vi "test13-AsteriskWildcardStateRegistration.vi"(8 "error in (no error)":errorcluster, 11 "TestCase in":refnum<class "testcase-CSMBroadcast.lvclass">) -> (0 "error out":errorcluster, 3 "TestCase out":refnum<class "testcase-CSMBroadcast.lvclass">)   [LabVIEW 2017, in "testcase-CSMBroadcast.lvclass"]
uses:
  testcase-CSMBroadcast.lvclass
  0c20cacf-7d77-4f8e-aec5-f22e7d09936d.vi
  2ac2ae3e-7b57-4584-ae51-4de7b8fb2940.vi
  26de337d-8090-412f-9da5-e117a55d4726.vi
  de10340a-d592-45ad-b055-7fa7b377c551.vi
  e3eae2f8-d8ce-4adb-8167-9a417250fce1.vi
  a4d00e00-a9ed-4631-bf53-269bf71f16fc.vi
  src/user.lib/_NEVSTOP/Communicable State Machine(CSM)/AdvanceAPI/CSM - Revert Arguments-Safe String.vi
  src/user.lib/_NEVSTOP/Communicable State Machine(CSM)/_Shared/Trim Single-line Text.vi
  src/user.lib/_NEVSTOP/Communicable State Machine(CSM)/AdvanceAPI/CSM - Make String Arguments Safe.vi
  src/user.lib/_NEVSTOP/Communicable State Machine(CSM)/AdvanceAPI/CSM - Break Down Multiple States String.vi
  src/user.lib/_NEVSTOP/Communicable State Machine(CSM)/AdvanceAPI/CSM - Compact Multiple States.vi
  src/user.lib/_NEVSTOP/Communicable State Machine(CSM)/AdvanceAPI/CSM - Keywords.vi
  src/user.lib/_NEVSTOP/Communicable State Machine(CSM)/AdvanceAPI/CSM - Set Module Attribute.vi
  src/user.lib/_NEVSTOP/Communicable State Machine(CSM)/AdvanceAPI/CSM - Get Module Attribute.vi
  <vilib>/addons/_JKI Toolkits/VI Tester/TestCase.llb/TestCase.lvclass
  src/user.lib/_NEVSTOP/Communicable State Machine(CSM)/Communicable State Machine.lvlib
  C:/Program Files (x86)/National Instruments/LabVIEW 2017/vi.lib/addons/_JKI Toolkits/VI Tester/TestCase.llb/TestCase.lvclass
panel:
  out "Execution Times":i32
  out "State History":string
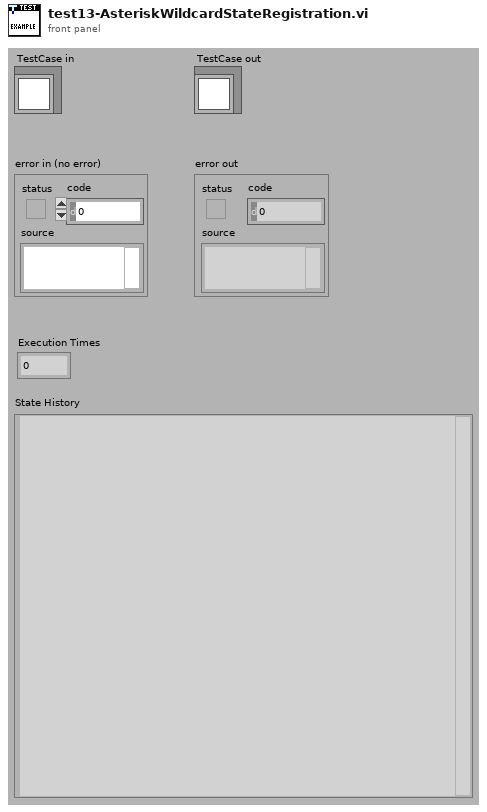
[diagram p1: front panel]
types:
  T1 = enum32{"Invalid", "Standard", "Closed", "Hidden", "Minimized", "Maximized"}
  T2 = enum32{"invalid app kind", "Development System", "Run Time System", "Student Edition", "Embedded LabVIEW", "Evaluation", "Custom"}
  T3 = typedef "Communicable State Machine.lvlib/_CSM_Response Source Message.ctl" = cluster{"‘State":string, "’Arguments":string, "’Error":errorcluster}
  T4 = cluster{"Current VI Reference":refnum<vi>, "Close Panel on Exit?":bool}
  T5 = cluster{"Core":cluster{"Current VI Reference":refnum<vi>, "Close Panel on Exit?":bool}, "Your Boolean data":bool, "Your string data":string, "TestData":i32}
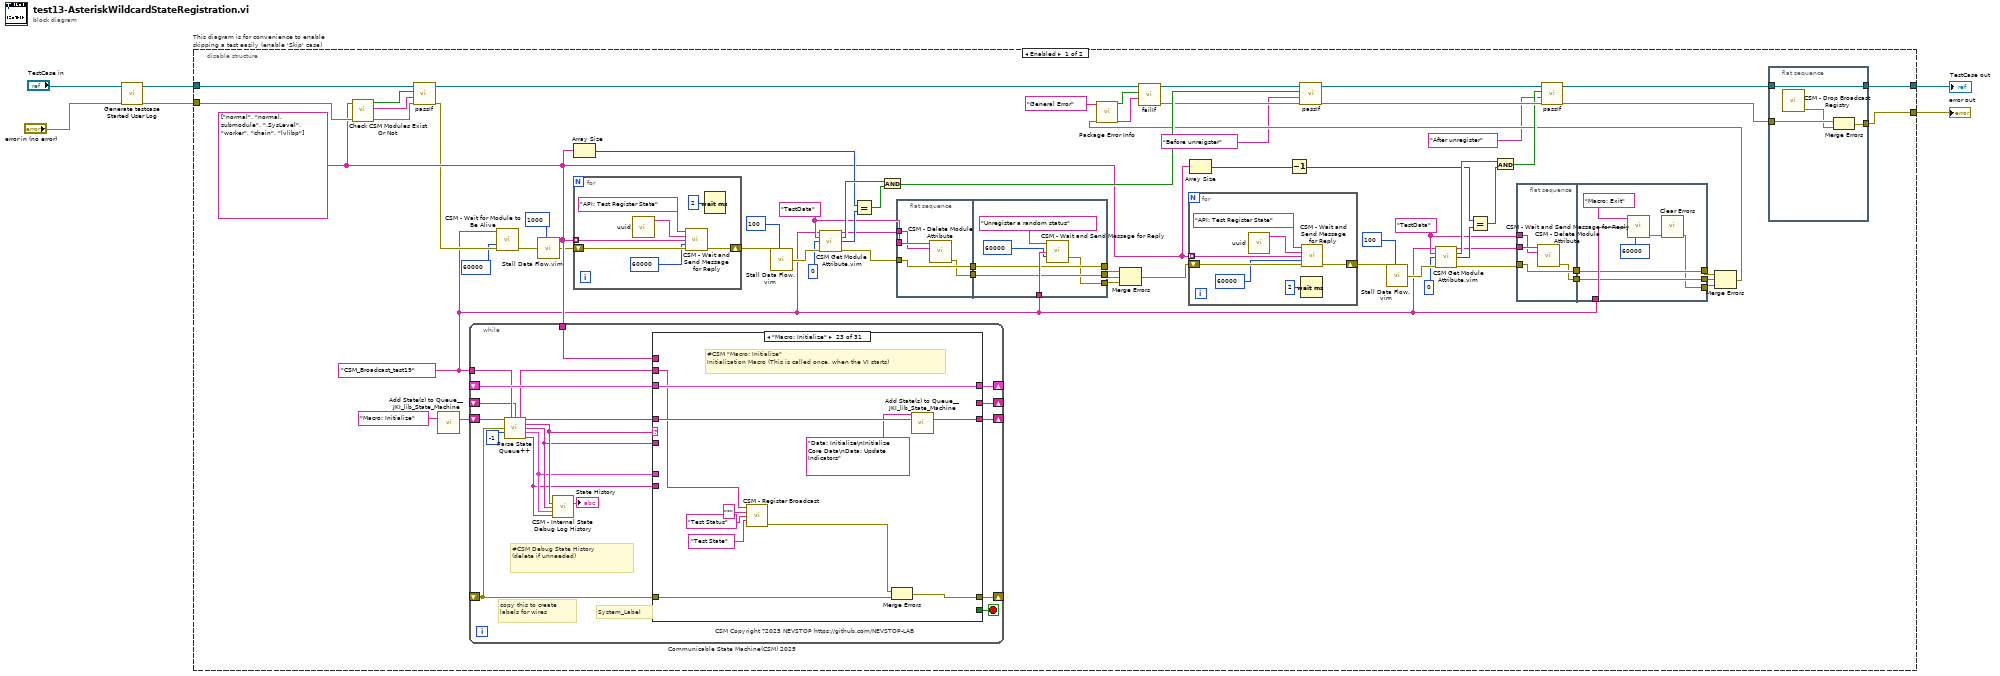
[diagram p0: block diagram]
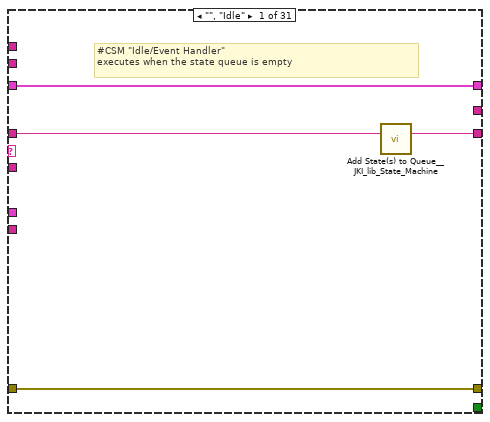
[diagram p2: hidden frame]
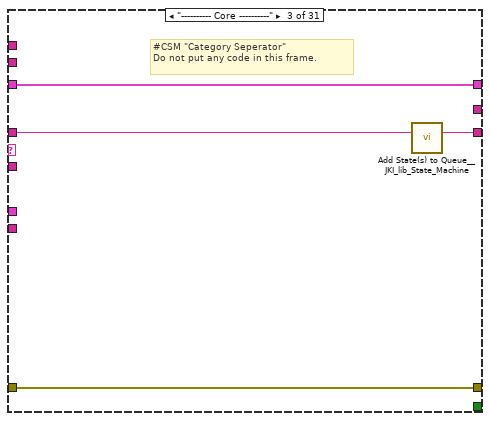
[diagram p4: hidden frame]
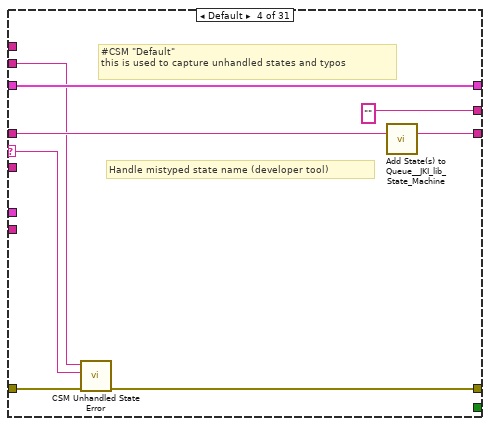
[diagram p5: hidden frame]
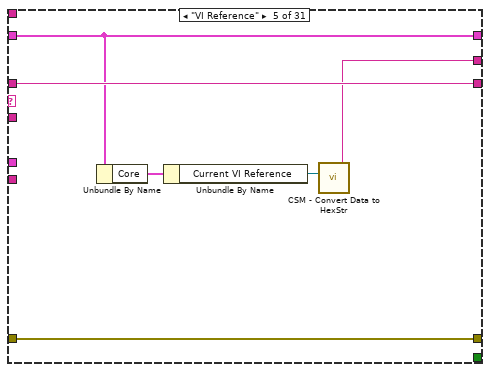
[diagram p6: hidden frame]
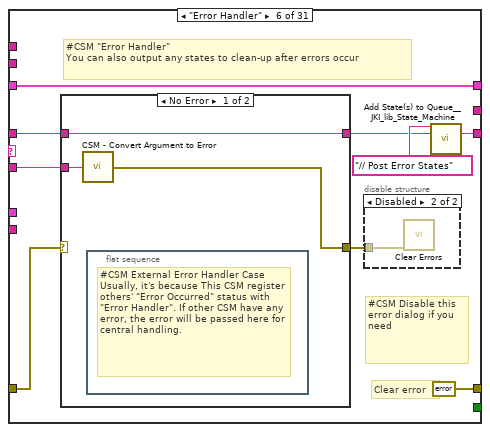
[diagram p7: hidden frame]
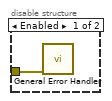
[diagram p8: hidden frame]
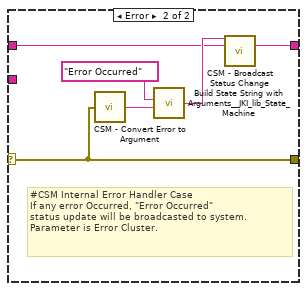
[diagram p9: hidden frame]
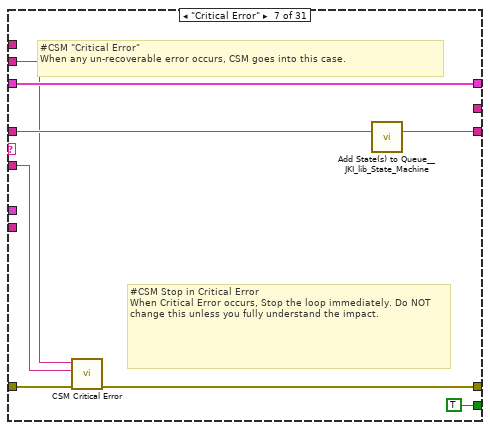
[diagram p10: hidden frame]
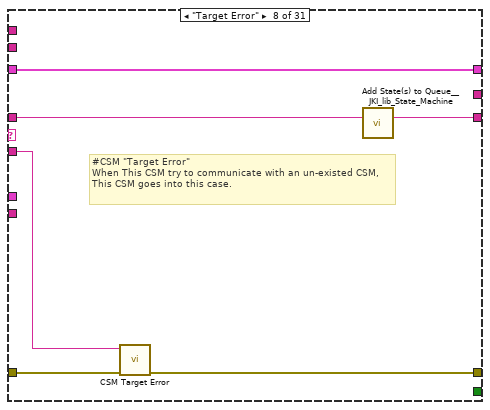
[diagram p11: hidden frame]
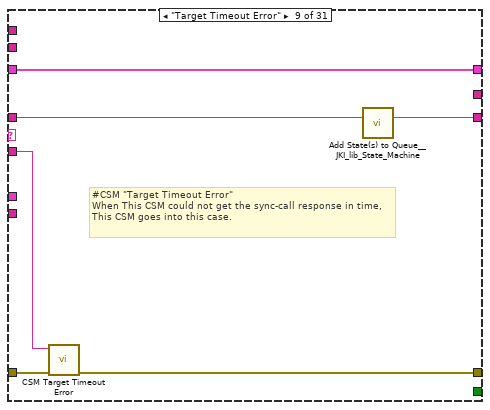
[diagram p12: hidden frame]
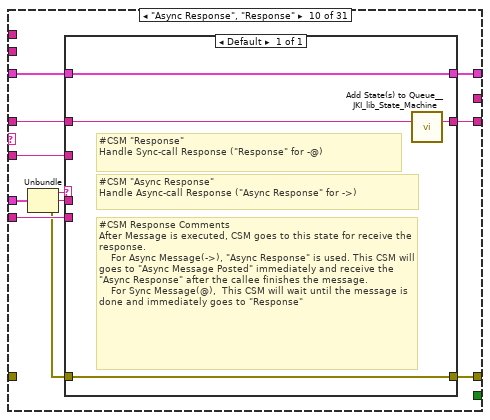
[diagram p13: hidden frame]
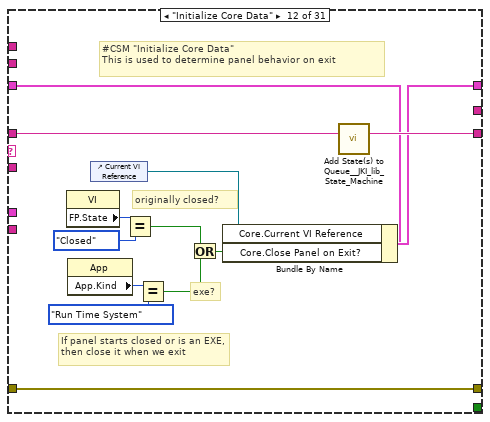
[diagram p15: hidden frame]
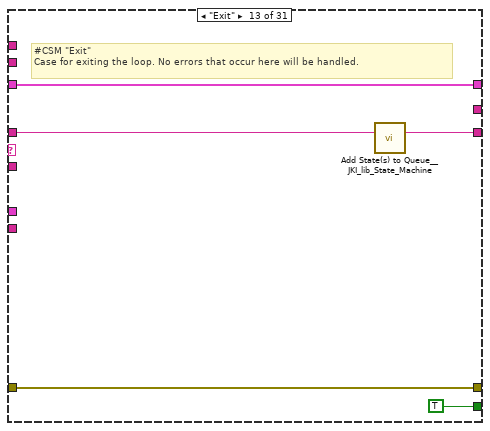
[diagram p16: hidden frame]
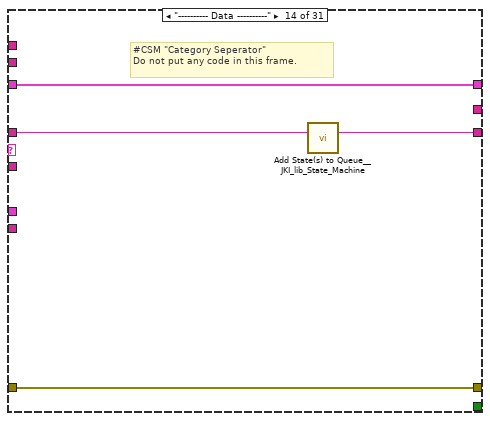
[diagram p17: hidden frame]
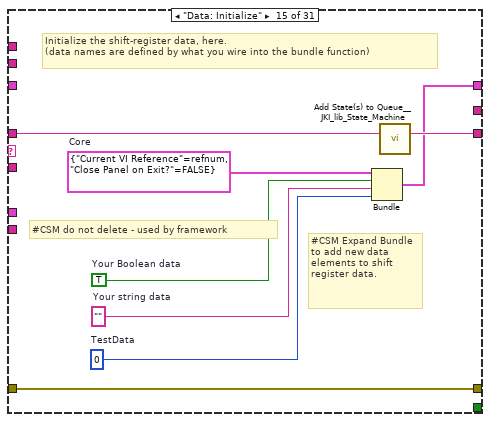
[diagram p18: hidden frame]
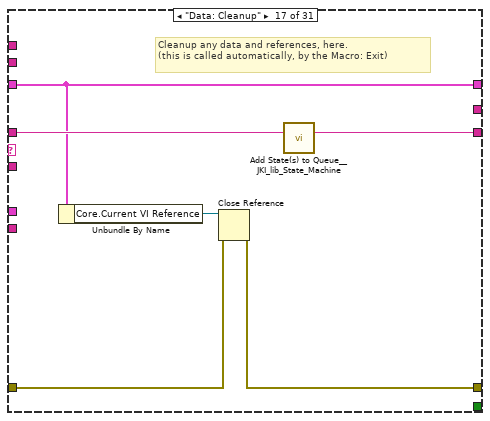
[diagram p20: hidden frame]
diagram:
  n1 = call "Generate testcase Started User Log.vi"("Error In"="error in (no error)") -> ("error out"=w1:errorcluster)  [unwired: 10 in]
  n2 = disable-structure "This diagram is for convenience to enable skipping a test easily (enable 'Skip' case)" shown="Enabled" {
    disable-tunnel: "TestCase in" -> [w27 w429]
    disable-tunnel: [w22 w427] -> w2
    disable-tunnel: [w21 w428] -> w4
    disable-tunnel: w1 -> [w26 w426]
    frame Enabled {
      w36 = "TestData" ("Attribute")
      w58 = "TestData" ("Attribute")
      w9 = "CSM_Broadcast_test19" ("Name (\"\" to Use UUID)")
      w25 = string[] ["normal", "normal.submodule", ".SysLevel", "worker", "chain", "lvlibp"]
      n3 = call "Check CSM Modules Exist Or Not.vi"("error in"=w26, "CSM names in"=w25) -> ("error out"=w28:errorcluster, "Debug string"=w29:string, "All Modules Exist?"=w30:bool)  [unwired: 7 in]
      n4 = call-dynamic "passIf.vi"("error in (no error)"=w28, "message (\"\")"=w29, "pass"=w30, "TestCase in"=w27) -> ("error out"=w10:errorcluster, "TestCase out"=w19:refnum<class "testcase-CSMBroadcast.lvclass">)  [unwired: 6 in]
      n5 = call <vilib>:"Add State(s) to Queue__JKI_lib_State_Machine.vi"("State(s) in (\"\")"="Macro: Initialize" ("Init State(\"Macro: Initialize\")")) -> ("States Out"=w69:string)  [unwired: 14 in]
      n6 = while "Communicable State Machine(CSM) 2025" {
        shift-right: [w116] -> _
        shift-left: _ -> [w115]
        shift-right: [w119] -> _
        shift-left: _ -> [w114]
        shift-right: [w118] -> _
        shift-left: w69 -> [w120]
        tunnel: w9 -> [w112]
        shift-right: [w113] -> _
        shift-left: _ -> [w106]
        tunnel: w25 -> [w103]
        stop <- w117 stop-if-true
        # "#CSM Debug State History\n(delete if unneeded)"
        # "copy this to create labels for wires"
        # "System_Label"
        # "CSM Copyright ?2025 NEVSTOP https://github.com/NEVSTOP-LAB"
        n7 = call "Parse State Queue++.vi"("State Queue"=w120, "Name (\"\" to Use UUID)"=w112, "Response Arguments"=w106, "Previous Error"=w114, "Dequeue (1 ms)"=-1 ("Timeout")) -> ("Name Used"=w107:string, "Remaining States"=w121:string, "Current State"=w111:string, "Arguments"=w110:string, "Additional Information"=w109:T3, "Source CSM"=w108:string)  [unwired: 5 in]
        n8 = call "CSM - Internal State Debug Log History.vi"("State"=w111, "Arguments (\"\")"=w110, ">> Response Source Message >>"=w109, "Source (\"\")"=w108) -> ("Debug Log"=→"State History":string)  [unwired: 11 in]
        n9 = case shown="\"Macro: Initialize\"" w111 {
          selector: w111 -> [_ _ _ w135 _ _ _ _ _ _ _ _ _ _ _ _ _ _ _ _ _ _ _ _ _ _ _ _ _ _ _]
          tunnel: w121 -> [w122 w127 w132 w139 w145 w151 w172 w178 w184 w192 w203 w217 w222 w226 w234 w236 w243 w247 w251 w257 w272 w341 w352 w365 w367 w371 w376 w383 w387 w398 w418]
          tunnel: w110 -> [_ _ _ _ _ w150 w168 w177 w182 w191 _ _ _ _ _ _ _ _ _ w252 w266 _ _ _ _ _ w374 _ _ _ _]
          tunnel: w115 -> [w123 w126 w129 w137 w144 w154 w173 w179 w185 w194 w202 w210 w220 w223 _ w235 w238 w244 w249 w255 w268 w338 w349 w362 w366 w370 w375 w380 w384 w390 w404]
          tunnel: [w124 w128 w130 w133 w146 errorcluster {"status"=FALSE, "code"=0, "source"=""} ("error out") w169 w175 w181 w197 w204 w214 w219 w224 w231 w237 w239 w245 w248 w253 w269 w339 w343 w354 w368 w372 w377 w381 w385 w392 w406] -> w119
          tunnel: w114 -> [w124 w128 w130 w140 w146 w152 w174 w176 w183 _ w204 w214 w219 w224 w231 w237 w240 w245 w248 w254 w270 w339 w350 w363 w368 w372 w377 w381 w385 w396 w416]
          tunnel: [w125 w127 w131 w138 w145 w147 w171 w180 w186 w193 w203 w216 w221 w225 w233 w236 w242 w246 w250 w256 w271 w340 w351 w364 w367 w371 w376 w382 w386 w397 w417] -> w118
          tunnel: [_ _ _ _ _ _ TRUE _ _ _ _ _ TRUE _ _ _ _ _ _ _ _ _ _ _ _ _ _ _ _ _ _] -> w117
          tunnel: [w123 w126 w129 w137 w144 w154 w173 w179 w185 w195 w202 w215 w220 w223 w232 w235 w238 w244 w249 w255 w268 w338 w349 w362 w366 w370 w375 w380 w384 w394 w402] -> w116
          tunnel: w108 -> [_ _ _ _ _ _ _ _ _ w189 _ _ _ _ _ _ _ _ _ _ _ _ _ _ _ _ _ _ _ _ _]
          tunnel: w109 -> [_ _ _ _ _ _ _ _ _ w196 _ _ _ _ _ _ _ _ _ _ _ _ _ _ _ _ _ _ _ _ _]
          tunnel: [_ _ _ "" w141 _ _ _ _ _ _ _ _ _ _ _ _ _ _ _ _ _ _ _ _ "API1 Response" w373 _ _ _ _] -> w113
          tunnel: w107 -> [_ _ _ w134 _ _ w167 _ _ _ _ _ _ _ _ _ _ _ _ _ _ _ w344 w356 _ _ _ _ _ w393 w413]
          tunnel: w103 -> [_ _ _ _ _ _ _ _ _ _ _ _ _ _ _ _ _ _ _ _ _ _ _ _ _ _ _ _ _ _ w409]
          frame "", "Idle" {
            # "#CSM \"Idle/Event Handler\"\nexecutes when the state queue is empty"
            n10 = call <vilib>:"Add State(s) to Queue__JKI_lib_State_Machine.vi"("State(s) in (\"\")"=w122) -> ("States Out"=w125:string)  [unwired: 14 in]
          }
          frame "CSM Documentation" {
            # "#CSM README FIRST\n\nCommunicable State Machine(CSM) is a LabVIEW application framework that builds upon JKI State Machine(JKISM). It follows the pattern of JKISM and extends the keywords to describe message communication between modules, including concepts such as Sync-Message, Async-Message, Subscription/Unsubscription of status - essential elements for creating reusable code modules. For more information, please visit the CSM wiki: https://nevstop-lab.github.io/CSM-Wiki/\n\nFor instructions on JKI State Machine, visit: http://jki.net/state-machine/\nFor information about CSM, visit: https://github.com/NEVSTOP-LAB"
            # "#CSM \"Documentation\"\nCase for holding CSM Documenation"
          }
          frame "---------- Core ----------" {
            # "#CSM \"Category Seperator\"\nDo not put any code in this frame."
            n11 = call <vilib>:"Add State(s) to Queue__JKI_lib_State_Machine.vi"("State(s) in (\"\")"=w132) -> ("States Out"=w131:string)  [unwired: 14 in]
          }
          frame Default {
            # "#CSM \"Default\"\nthis is used to capture unhandled states and typos"
            # "Handle mistyped state name (developer tool)"
            n12 = call "CSM Unhandled State Error.vi"("error in (no error)"=w140, "Undefined State"=w135, "CSM Name"=w134) -> ("error out"=w133:errorcluster)  [unwired: 8 in]
            n13 = call <vilib>:"Add State(s) to Queue__JKI_lib_State_Machine.vi"("State(s) in (\"\")"=w139) -> ("States Out"=w138:string)  [unwired: 14 in]
          }
          frame "VI Reference" {
            n14 = Unbundle By Name(w144) -> ("Core"=w143:T4)
            n15 = Unbundle By Name(w143) -> ("Current VI Reference"=w142:refnum<vi>)
            n16 = call "CSM - Convert Data to HexStr.vi"("Variant"=w142) -> ("HEX String (0-9,A-F)"=w141:string)  [unwired: 8 in]
          }
          frame "Error Handler" {
            # "#CSM Disable this error dialog if you need"
            # "#CSM \"Error Handler\"\nYou can also output any states to clean-up after errors occur"
            # "Clear error"
            n17 = case shown="No Error" w152 {
              selector: w152 -> [_ w161]
              tunnel: [w160 w163] -> w148
              tunnel: w151 -> [w160 w162]
              tunnel: w150 -> [w159 _]
              tunnel: [w158 w161] -> w153
              frame No Error {
                n18 = call "CSM - Convert Argument to Error.vi"("Argument"=w159) -> ("Error"=w158:errorcluster)  [unwired: 4 in]
                n19 = flat-sequence {
                  frame #0 {
                    # "#CSM External Error Handler Case\nUsually, it's because This CSM register others' \"Error Occurred\" status with \"Error Handler\". If other CSM have any error, the error will be passed here for central handling."
                  }
                }
              }
              frame Error {
                # "#CSM Internal Error Handler Case \nIf any error Occurred, \"Error Occurred\" \nstatus update will be broadcasted to system.\nParameter is Error Cluster."
                n20 = call "CSM - Convert Error to Argument.vi"("Error"=w161) -> ("Argument"=w165:string)  [unwired: 4 in]
                n21 = call <vilib>:"Build State String with Arguments__JKI_lib_State_Machine.vi"("Arguments (\"\")"=w165, "State"="Error Occurred" ("Status with Arguments")) -> ("State with Arguments"=w164:string)  [unwired: 4 in]
                n22 = call "CSM - Broadcast Status Change.vi"("Status With Arguments"=w164, "State Queue"=w162) -> ("Remaining States"=w163:string)  [unwired: 13 in]
              }
            }
            n23 = disable-structure shown="Disabled" {
              disable-tunnel: w153 -> [w156 w157]
              frame Enabled {
                n24 = call <vilib>:"General Error Handler.vi"("error in (no error)"=w156) -> ()  [unwired: 10 in, 5 out]
              }
              frame Disabled {
                n25 = call <vilib>:"Clear Errors.vi"("error in (no error)"=w157) -> ()  [unwired: 5 in, 2 out]
              }
            }
            n26 = call <vilib>:"Add State(s) to Queue__JKI_lib_State_Machine.vi"("State(s) in Front (\"\")"="// Post Error States", "State(s) in (\"\")"=w148) -> ("States Out"=w147:string)  [unwired: 13 in]
          }
          frame "Critical Error" {
            # "#CSM Stop in Critical Error\nWhen Critical Error occurs, Stop the loop immediately. Do NOT change this unless you fully understand the impact."
            # "#CSM \"Critical Error\"\nWhen any un-recoverable error occurs, CSM goes into this case."
            n27 = call "CSM Critical Error.vi"("error in (no error)"=w174, "Arugments (As Reason)"=w168, "CSM Name"=w167) -> ("error out"=w169:errorcluster)  [unwired: 8 in]
            n28 = call <vilib>:"Add State(s) to Queue__JKI_lib_State_Machine.vi"("State(s) in (\"\")"=w172) -> ("States Out"=w171:string)  [unwired: 14 in]
          }
          frame "Target Error" {
            # "#CSM \"Target Error\"\nWhen This CSM try to communicate with an un-existed CSM, This CSM goes into this case."
            n29 = call "CSM Target Error.vi"("error in (no error)"=w176, "Arguments (As CSM Name)"=w177) -> ("error out"=w175:errorcluster)  [unwired: 9 in]
            n30 = call <vilib>:"Add State(s) to Queue__JKI_lib_State_Machine.vi"("State(s) in (\"\")"=w178) -> ("States Out"=w180:string)  [unwired: 14 in]
          }
          frame "Target Timeout Error" {
            # "#CSM \"Target Timeout Error\"\nWhen This CSM could not get the sync-call response in time, This CSM goes into this case."
            n31 = call "CSM Target Timeout Error.vi"("error in (no error)"=w183, "Arguments (As CSM Name)"=w182) -> ("error out"=w181:errorcluster)  [unwired: 9 in]
            n32 = call <vilib>:"Add State(s) to Queue__JKI_lib_State_Machine.vi"("State(s) in (\"\")"=w184) -> ("States Out"=w186:string)  [unwired: 14 in]
          }
          frame "Async Response", "Response" {
            n33 = Unbundle(w196) -> ("‘State"=w190:string, "’Arguments"=w188:string, "’Error"=w187:errorcluster)
            n34 = case shown="Default" w190 {
              tunnel: [w201] -> w197
              tunnel: w187 -> [w201]
              tunnel: [w200] -> w195
              tunnel: w194 -> [w200]
              tunnel: [w198] -> w193
              tunnel: w192 -> [w199]
              tunnel: w191 -> [_]
              tunnel: w189 -> [_]
              tunnel: w188 -> [_]
              frame Default {
                # "#CSM Response Comments\nAfter Message is executed, CSM goes to this state for receive the response.\n    For Async Message(->), \"Async Response\" is used. This CSM will goes to \"Async Message Posted\" immediately and receive the \"Async Response\" after the callee finishes the message.\n    For Sync Message(@),  This CSM will wait until the message is done and immediately goes to \"Response\""
                # "#CSM \"Async Response\"\nHandle Async-call Response (\"Async Response\" for ->)"
                # "#CSM \"Response\"\nHandle Sync-call Response (\"Response\" for -@)"
                n35 = call <vilib>:"Add State(s) to Queue__JKI_lib_State_Machine.vi"("State(s) in (\"\")"=w199) -> ("States Out"=w198:string)  [unwired: 14 in]
              }
            }
          }
          frame "Async Message Posted" {
            # "#CSM \"Async Message Posted\"\nAfter Async Message is posted (-> or ->| ), CSM goes to this state for post-action.\nYou can use Argument - State to tell which Async Message is called."
          }
          frame "Initialize Core Data" {
            # "#CSM \"Initialize Core Data\"\nThis is used to determine panel behavior on exit"
            # "originally closed?"
            # "exe?"
            # "If panel starts closed or is an EXE, then close it when we exit"
            n36 = property class="VI"() -> ("FP.State"=w207:T1)  [unwired: 2 in, 2 out]
            n37 = property class="App"() -> ("App.Kind"=w213:T2)  [unwired: 2 in, 2 out]
            n38 = control-ref of="Current VI Reference"() -> (w208:refnum<vi>)
            n39 = Equal?(x=w207, y=T1."Closed" ("Front Panel Window:State")) -> (x = y?=w205:bool)
            n40 = Equal?(x=w213, y=T2."Run Time System" ("Application:Kind")) -> (x = y?=w211:bool)
            n41 = Or(x=w205, y=w211) -> (x .or. y?=w209:bool)
            n42 = Bundle By Name(cluster=w210, "Core.Current VI Reference"=w208, "Core.Close Panel on Exit?"=w209) -> (w215:T5)
            n43 = call <vilib>:"Add State(s) to Queue__JKI_lib_State_Machine.vi"("State(s) in (\"\")"=w217) -> ("States Out"=w216:string)  [unwired: 14 in]
          }
          frame "Exit" {
            # "#CSM \"Exit\"\nCase for exiting the loop. No errors that occur here will be handled."
            n44 = call <vilib>:"Add State(s) to Queue__JKI_lib_State_Machine.vi"("State(s) in (\"\")"=w222) -> ("States Out"=w221:string)  [unwired: 14 in]
          }
          frame "---------- Data ----------" {
            # "#CSM \"Category Seperator\"\nDo not put any code in this frame."
            n45 = call <vilib>:"Add State(s) to Queue__JKI_lib_State_Machine.vi"("State(s) in (\"\")"=w226) -> ("States Out"=w225:string)  [unwired: 14 in]
          }
          frame "Data: Initialize" {
            w227 = 0  # TestData
            w228 = T4 {"Current VI Reference"=refnum, "Close Panel on Exit?"=FALSE}  # Core
            w230 = TRUE  # Your Boolean data
            w229 = ""  # Your string data
            # "#CSM do not delete - used by framework"
            # "#CSM Expand Bundle to add new data elements to shift register data."
            # "Initialize the shift-register data, here.\n(data names are defined by what you wire into the bundle function)"
            n46 = Bundle("Core"=w228, "Your Boolean data"=w230, "Your string data"=w229, "TestData"=w227) -> (w232:T5)  [unwired: 1 in]
            n47 = call <vilib>:"Add State(s) to Queue__JKI_lib_State_Machine.vi"("State(s) in (\"\")"=w234) -> ("States Out"=w233:string)  [unwired: 14 in]
          }
          frame "Data: Update Indicators" {
          }
          frame "Data: Cleanup" {
            # "Cleanup any data and references, here.\n(this is called automatically, by the Macro: Exit)"
            n48 = Unbundle By Name(w238) -> ("Core.Current VI Reference"=w241:refnum<vi>)
            n49 = Close Reference(reference=w241, error in (no error)=w240) -> (error out=w239:errorcluster)
            n50 = call <vilib>:"Add State(s) to Queue__JKI_lib_State_Machine.vi"("State(s) in (\"\")"=w243) -> ("States Out"=w242:string)  [unwired: 14 in]
          }
          frame "---------- UI ----------" {
            # "#CSM \"Category Seperator\"\nDo not put any code in this frame."
            n51 = call <vilib>:"Add State(s) to Queue__JKI_lib_State_Machine.vi"("State(s) in (\"\")"=w247) -> ("States Out"=w246:string)  [unwired: 14 in]
          }
          frame "UI: Initialize" {
            # "#CSM \"UI: Initialize\"\nInitialize the User Interface, here.\n(this is called automatically, by the Macro: Init)"
            n52 = call <vilib>:"Add State(s) to Queue__JKI_lib_State_Machine.vi"("State(s) in (\"\")"=w251) -> ("States Out"=w250:string)  [unwired: 14 in]
          }
          frame "UI: Cursor Set" {
            # "#CSM \"UI: Cursor Set\"\nSet and Unset Cursor Busy.\n(Usage: \"UI: Cursor Set >> Busy|Idle\")"
            # "Argument"
            n53 = disable-structure shown="TARGET_TYPE!=Windows" {
              disable-tunnel: w254 -> [w260 w265]
              disable-tunnel: [w259 w265] -> w253
              disable-tunnel: w252 -> [w258 _]
              frame condition #0 (active) {
                n54 = case shown="\"Idle\", Default" w258 {
                  tunnel: w260 -> [w262 w264]
                  tunnel: [w261 w263] -> w259
                  frame "Idle", Default {
                    n55 = call <vilib>:"Unset Busy.vi"("error in (no error)"=w262) -> ("error out"=w261:errorcluster)  [unwired: 10 in]
                  }
                  frame "Busy" {
                    n56 = call <vilib>:"Set Busy.vi"("error in (no error)"=w264) -> ("error out"=w263:errorcluster)  [unwired: 9 in, 1 out]
                  }
                }
              }
              frame condition #1 {
              }
            }
            n57 = call <vilib>:"Add State(s) to Queue__JKI_lib_State_Machine.vi"("State(s) in (\"\")"=w257) -> ("States Out"=w256:string)  [unwired: 14 in]
          }
          frame "UI: Front Panel State" {
            # "#CSM \"UI: Front Panel State\"\nSet Front Panel Open or Closed\n(Usage: \"UI: Front Panel State >> Open|Close\")"
            # "Argument"
            n58 = Unbundle By Name(w268) -> ("Core.Current VI Reference"=w267:refnum<vi>)
            n59 = call <vilib>:"Add State(s) to Queue__JKI_lib_State_Machine.vi"("State(s) in (\"\")"=w272) -> ("States Out"=w271:string)  [unwired: 14 in]
            n60 = case shown="\"Close\", \"Closed\"" w266 {
              tunnel: w270 -> [w278 w293 w304 w317 w330]
              tunnel: [w280 w294 w306 w319 w332] -> w269
              tunnel: w267 -> [w279 w291 w305 w318 w331]
              frame "Open", "Standard", Default {
                w273 = T1."Standard" ("State")
                n61 = property class="VI"(reference=w279, error in=w278) -> (reference out=w276:refnum<vi>, error out=w277:errorcluster, "FP.State"=w275:T1)
                n62 = Not Equal?(x=w275, y=w273) -> (x != y?=w274:bool)
                n63 = case shown="True" w274 {
                  tunnel: [w284 w286] -> w280
                  tunnel: w277 -> [w283 w286]
                  tunnel: w276 -> [w282 _]
                  tunnel: w273 -> [w281 _]
                  frame True {
                    n64 = invoke class="VI" method="FP.Open"(reference=w282, error in=w283, "Activate"=TRUE, "State"=w281) -> (error out=w284:errorcluster)  [unwired: 1 in, 4 out]
                  }
                  frame False {
                  }
                }
              }
              frame "Close", "Closed" {
                n65 = property class="VI"(reference=w291, error in=w293) -> (reference out=w290:refnum<vi>, error out=w292:errorcluster, "FP.State"=w288:T1)
                n66 = Not Equal?(x=w288, y=T1."Closed" ("Front Panel Window:State")) -> (x != y?=w287:bool)
                n67 = case shown="False" w287 {
                  tunnel: [w295 w298] -> w294
                  tunnel: w292 -> [w295 w297]
                  tunnel: w290 -> [_ w296]
                  frame False {
                  }
                  frame True {
                    n68 = invoke class="VI" method="FP.Close"(reference=w296, error in=w297) -> (error out=w298:errorcluster)  [unwired: 1 in, 2 out]
                  }
                }
              }
              frame "Hidden", "Hide" {
                w299 = T1."Hidden" ("State")
                n69 = property class="VI"(reference=w305, error in=w304) -> (reference out=w302:refnum<vi>, error out=w303:errorcluster, "FP.State"=w301:T1)
                n70 = Not Equal?(x=w301, y=w299) -> (x != y?=w300:bool)
                n71 = case shown="True" w300 {
                  tunnel: [w310 w311] -> w306
                  tunnel: w303 -> [w309 w311]
                  tunnel: w302 -> [w308 _]
                  tunnel: w299 -> [w307 _]
                  frame True {
                    n72 = invoke class="VI" method="FP.Open"(reference=w308, error in=w309, "State"=w307) -> (error out=w310:errorcluster)  [unwired: 2 in, 4 out]
                  }
                  frame False {
                  }
                }
              }
              frame "Minimize", "Minimized" {
                w312 = T1."Minimized" ("State")
                n73 = property class="VI"(reference=w318, error in=w317) -> (reference out=w315:refnum<vi>, error out=w316:errorcluster, "FP.State"=w314:T1)
                n74 = Not Equal?(x=w314, y=w312) -> (x != y?=w313:bool)
                n75 = case shown="True" w313 {
                  tunnel: [w323 w324] -> w319
                  tunnel: w316 -> [w322 w324]
                  tunnel: w315 -> [w321 _]
                  tunnel: w312 -> [w320 _]
                  frame True {
                    n76 = invoke class="VI" method="FP.Open"(reference=w321, error in=w322, "State"=w320) -> (error out=w323:errorcluster)  [unwired: 2 in, 4 out]
                  }
                  frame False {
                  }
                }
              }
              frame "Maximize", "Maximized" {
                w325 = T1."Maximized" ("State")
                n77 = property class="VI"(reference=w331, error in=w330) -> (reference out=w328:refnum<vi>, error out=w329:errorcluster, "FP.State"=w327:T1)
                n78 = Not Equal?(x=w327, y=w325) -> (x != y?=w326:bool)
                n79 = case shown="True" w326 {
                  tunnel: [w336 w337] -> w332
                  tunnel: w329 -> [w335 w337]
                  tunnel: w328 -> [w334 _]
                  tunnel: w325 -> [w333 _]
                  frame True {
                    n80 = invoke class="VI" method="FP.Open"(reference=w334, error in=w335, "State"=w333) -> (error out=w336:errorcluster)  [unwired: 2 in, 4 out]
                  }
                  frame False {
                  }
                }
              }
            }
          }
          frame "---------- Macro ----------" {
            # "#CSM \"Category Seperator\"\nDo not put any code in this frame."
            n81 = call <vilib>:"Add State(s) to Queue__JKI_lib_State_Machine.vi"("State(s) in (\"\")"=w341) -> ("States Out"=w340:string)  [unwired: 14 in]
          }
          frame "Macro: Initialize" {
            # "#CSM \"Macro: Initialize\"\nInitialization Macro (This is called once, when the VI starts)"
            n82 = call "CSM - Register Broadcast.vi"("CSM Name(Empty for Broadcast Event)"=w344, "Source CSM Name (* as Default)"="*", "Trigger"="Test Status" ("Status"), "API (If \"\", Same as Trigger)"="Test State" ("Response Message (If \"\", Same as Source Message)")) -> ("error out"=w342:errorcluster)  [unwired: 10 in, 1 out]
            n83 = Merge Errors(w342, w350) -> (w343:errorcluster)
            n84 = call <vilib>:"Add State(s) to Queue__JKI_lib_State_Machine.vi"("State(s) in Front (\"\")"="Data: Initialize\nInitialize Core Data\nData: Update Indicators", "State(s) in (\"\")"=w352) -> ("States Out"=w351:string)  [unwired: 13 in]
          }
          frame "Macro: Exit" {
            # "#CSM \"Macro: Exit\"\nExit Macro (This is called once, when the VI exits)"
            n85 = call "CSM - Unregister Broadcast.vi"("CSM Name(Empty for Broadcast Event)"=w356, "Source CSM Name (* as Default)"="*", "Trigger"="Test Status" ("Status"), "API (\"*\" as Default)"="Test State" ("Response Message (If \"\", Same as Source Message)")) -> ("error out"=w353:errorcluster)  [unwired: 10 in, 1 out]
            n86 = call <vilib>:"Add State(s) to Queue__JKI_lib_State_Machine.vi"("State(s) in Front (\"\")"="//Exit Sub-Modules ", "State(s) at Back (\"\")"="Data: Cleanup\nExit") -> ("States Out"=w360:string)  [unwired: 13 in]
            n87 = Merge Errors(w353, w363) -> (w354:errorcluster)
            n88 = call <vilib>:"Add State(s) to Queue__JKI_lib_State_Machine.vi"("State(s) in Front (\"\")"=w360, "State(s) in (\"\")"=w365) -> ("States Out"=w364:string)  [unwired: 13 in]
          }
          frame "---------- API ----------" {
            # "#CSM \"Category Seperator\"\nDo not put any code in this frame."
          }
          frame "API: API1" {
            # "#CSM API Example\nCopy/Rename this case for your own API"
            # "#CSM Response\nConnect this to return the response of your API"
            # "#CSM >> Msg/Rep's CSM >>\nIf you need to tell who triggered this state , use this string. If it's this case itself, this string is \"\"."
            # "#CSM >> Arguments >>\nDeal with the parameter if any"
          }
          frame "API: API2" {
            # "#CSM API Example\nCopy/Rename this case for your own API"
            # "unpack Hex String  to Variant\nif complex parameter is needed."
            n89 = call "CSM - Convert HexStr to Data.vi"("HEX String"=w374) -> ()  [unwired: 7 in, 2 out]
            n90 = disable-structure shown="Disabled" {
              disable-tunnel: [w378 "API2 Response"] -> w373
              frame Disabled {
                # "pack variant to hexstr \nif complex response is needed."
                # "complex Response"
                n91 = call "CSM - Convert Data to HexStr.vi"() -> ("HEX String (0-9,A-F)"=w378:string)  [unwired: 9 in]
              }
              frame Enabled {
              }
            }
          }
          frame "---------- Action ----------" {
            # "#CSM \"Category Seperator\"\nDo not put any code in this frame."
            n92 = call <vilib>:"Add State(s) to Queue__JKI_lib_State_Machine.vi"("State(s) in (\"\")"=w383) -> ("States Out"=w382:string)  [unwired: 14 in]
          }
          frame "Action: action1" {
            # "#CSM \"Internal State\"\nThis category is used for holding internal states"
            n93 = call <vilib>:"Add State(s) to Queue__JKI_lib_State_Machine.vi"("State(s) in (\"\")"=w387) -> ("States Out"=w386:string)  [unwired: 14 in]
          }
          frame "Test State" {
            n94 = Unbundle By Name(w390) -> ("TestData"=w395:i32)
            n95 = disable-structure shown="Enabled" {
              frame Disabled {
                n96 = feedback #1(0 ("y")) -> (w400:i32)
                n97 = Increment(x=w400) -> (x+1=w399:i32)
                "Execution Times" <- w399
                n98 = feedback-in #1(w399) -> ()
              }
              frame Enabled {
              }
            }
            n99 = Increment(x=w395) -> (x+1=w388:i32)
            n100 = Bundle By Name(cluster=w390, "TestData"=w388) -> (w394:T5)
            n101 = call "CSM Set Module Attribute.vim"("CSM Name"=w393, "Attribute"="TestData", "Value"=w388) -> ("error out"=w391:errorcluster)  [unwired: 9 in, 3 out]
            n102 = call <vilib>:"Add State(s) to Queue__JKI_lib_State_Machine.vi"("State(s) in (\"\")"=w398) -> ("States Out"=w397:string)  [unwired: 14 in]
            n103 = Merge Errors(w396, w391) -> (w392:errorcluster)
          }
          frame "Unregister a random status" {
            n104 = Random Number (0-1)() -> (number: 0 to 1=w411:dbl)
            n105 = Array Size(array=w409) -> (size(s)=w412:i32)
            n106 = Multiply(x=w412, y=w411) -> (x*y=w410:dbl)
            n107 = Bundle By Name(cluster=w404, "TestData"=0) -> (w402:T5)
            n108 = Round Toward -Infinity(1:w410) -> (0:w408:dbl)
            n109 = Index Array(array=w409, index=w408) -> (element=w407:string)
            n110 = call "CSM - Unregister Broadcast.vi"("CSM Name(Empty for Broadcast Event)"=w413, "Source CSM Name (* as Default)"=w407, "Trigger"="Test Status" ("Status"), "API (\"*\" as Default)"="Test State" ("Response Message (If \"\", Same as Source Message)")) -> ("error out"=w405:errorcluster)  [unwired: 10 in, 1 out]
            n111 = Merge Errors(w416, w405) -> (w406:errorcluster)
            n112 = call <vilib>:"Add State(s) to Queue__JKI_lib_State_Machine.vi"("State(s) in (\"\")"=w418) -> ("States Out"=w417:string)  [unwired: 14 in]
          }
        }
      }
      n113 = call "CSM - Wait for Module to Be Alive.vi"("CSM Name"=w9, "Wait (5000 ms)"=60000, "error in (no error)"=w10) -> ("error out"=w11:errorcluster)  [unwired: 10 in, 2 out]
      n114 = call "Stall Data Flow.vim"("value in"=w11, "milliseconds to wait"=u32 1000) -> ("value out"=w7:errorcluster)  [unwired: 1 out]
      n115 = for {
        tunnel: w25 -> [w423] mode=indexing
        shift-right: [w422] -> w67
        shift-left: w7 -> [w421]
        n116 = call "uuid.vi"() -> ("UUID"=w424:string)  [unwired: 11 in]
        n117 = call "CSM - Wait and Send Message for Reply.vi"("State"="API: Test Register State", "Arguments (\"\")"=w424, "Target Module"=w423, "Wait (5000ms)"=60000, "Error In (No Error)"=w421) -> ("error out"=w422:errorcluster)  [unwired: 7 in, 3 out]
        n118 = Wait (ms)(milliseconds to wait=u32 2) -> ()  [unwired: 1 out]
      }
      n119 = Array Size(array=w25) -> (size(s)=w62:i32)
      n120 = call "Stall Data Flow.vim"("value in"=w67, "milliseconds to wait"=u32 100) -> ("value out"=w66:errorcluster)  [unwired: 1 out]
      n121 = call "CSM Get Module Attribute.vim"("CSM Name"=w9, "Attribute"=w58, "Default Value (Empty Variant)"=0 ("x+1"), "Error In"=w66) -> ("CSM Name (Dup)"=w59:string, "Found"=w64:bool, "Value"=w63:i32, "error out"=w57:errorcluster)  [unwired: 7 in, 1 out]
      n122 = Equal?(x=w62, y=w63) -> (x = y?=w61:bool)
      n123 = And(x=w64, y=w61) -> (x .and. y?=w60:bool)
      n124 = flat-sequence {
        tunnel: w59 -> [w96]
        tunnel: w58 -> [w95]
        tunnel: w57 -> [w94]
        tunnel: [w94] -> w56
        tunnel: [w93] -> w55
        tunnel: w9 -> [w101]
        tunnel: w56 -> [w100]
        tunnel: w55 -> [w99]
        tunnel: [w100] -> w54
        tunnel: [w99] -> w53
        tunnel: [w98] -> w52
        frame #0 {
          n125 = call "CSM - Delete Module Attribute.vi"("CSM Name"=w96, "Attribute"=w95) -> ("error out"=w93:errorcluster)  [unwired: 10 in, 3 out]
        }
        frame #1 {
          n126 = call "CSM - Wait and Send Message for Reply.vi"("State"="Unregister a random status", "Target Module"=w101, "Wait (5000ms)"=60000) -> ("error out"=w98:errorcluster)  [unwired: 9 in, 3 out]
        }
      }
      n127 = Merge Errors(w54, w53, w52) -> (w44:errorcluster)
      n128 = for {
        tunnel: w25 -> [w90] mode=indexing
        shift-right: [w89] -> w50
        shift-left: w44 -> [w88]
        n129 = call "uuid.vi"() -> ("UUID"=w91:string)  [unwired: 11 in]
        n130 = Wait (ms)(milliseconds to wait=u32 2) -> ()  [unwired: 1 out]
        n131 = call "CSM - Wait and Send Message for Reply.vi"("State"="API: Test Register State", "Arguments (\"\")"=w91, "Target Module"=w90, "Wait (5000ms)"=60000, "Error In (No Error)"=w88) -> ("error out"=w89:errorcluster)  [unwired: 7 in, 3 out]
      }
      n132 = Array Size(array=w25) -> (size(s)=w43:i32)
      n133 = Decrement(x=w43) -> (x-1=w42:i32)
      n134 = call "Stall Data Flow.vim"("value in"=w50, "milliseconds to wait"=u32 100) -> ("value out"=w49:errorcluster)  [unwired: 1 out]
      n135 = call "CSM Get Module Attribute.vim"("CSM Name"=w9, "Attribute"=w36, "Default Value (Empty Variant)"=0 ("x+1"), "Error In"=w49) -> ("CSM Name (Dup)"=w37:string, "Found"=w47:bool, "Value"=w46:i32, "error out"=w35:errorcluster)  [unwired: 7 in, 1 out]
      n136 = Equal?(x=w42, y=w46) -> (x = y?=w45:bool)
      n137 = And(x=w47, y=w45) -> (x .and. y?=w31:bool)
      n138 = flat-sequence {
        tunnel: w37 -> [w78]
        tunnel: w36 -> [w77]
        tunnel: w35 -> [w76]
        tunnel: [w76] -> w39
        tunnel: [w75] -> w38
        tunnel: w9 -> [w84]
        tunnel: w39 -> [w83]
        tunnel: w38 -> [w82]
        tunnel: [w83] -> w34
        tunnel: [w82] -> w33
        tunnel: [w80] -> w32
        frame #0 {
          n139 = call "CSM - Delete Module Attribute.vi"("CSM Name"=w78, "Attribute"=w77) -> ("error out"=w75:errorcluster)  [unwired: 10 in, 3 out]
        }
        frame #1 {
          n140 = call "CSM - Wait and Send Message for Reply.vi"("State"="Macro: Exit", "Target Module"=w84, "Response Timeout (-2 Using Global Settings)"=60000) -> ("error out"=w81:errorcluster)  [unwired: 9 in, 3 out]
          n141 = call <vilib>:"Clear Errors.vi"("error in (no error)"=w81) -> ("error out"=w80:errorcluster)  [unwired: 5 in, 1 out]
        }
      }
      n142 = Merge Errors(w34, w33, w32) -> (w15:errorcluster)
      n143 = call "Package Error Info.vi"("error in"=w15, "String in"="General Error") -> ("packed error info out"=w16:string, "error status"=w20:bool)  [unwired: 8 in]
      n144 = call-dynamic "failIf.vi"("message (\"\")"=w16, "fail"=w20, "TestCase in"=w19) -> ("error out"=w17:errorcluster, "TestCase out"=w18:refnum<class "testcase-CSMBroadcast.lvclass">)  [unwired: 7 in]
      n145 = call-dynamic "passIf.vi"("error in (no error)"=w17, "message (\"\")"="Before unreigster" ("message (\"\")"), "pass"=w60, "TestCase in"=w18) -> ("error out"=w41:errorcluster, "TestCase out"=w40:refnum<class "testcase-CSMBroadcast.lvclass">)  [unwired: 6 in]
      n146 = call-dynamic "passIf.vi"("error in (no error)"=w41, "message (\"\")"="After unregister" ("message (\"\")"), "pass"=w31, "TestCase in"=w40) -> ("error out"=w23:errorcluster, "TestCase out"=w24:refnum<class "testcase-CSMBroadcast.lvclass">)  [unwired: 6 in]
      n147 = flat-sequence {
        tunnel: w23 -> [w74]
        tunnel: [w73] -> w21
        tunnel: w24 -> [w71]
        tunnel: [w71] -> w22
        frame #0 {
          n148 = call "CSM - Drop Broadcast Registry.vi"() -> ("error out"=w72:errorcluster)  [unwired: 15 in]
          n149 = Merge Errors(w74, w72) -> (w73:errorcluster)
        }
      }
    }
    frame Disabled {
      # "skip test result while test is under development"
      n150 = call <vilib>:"skip.vi"("error in (no error)"=w426, "TestCase in"=w429) -> ("error out"=w428:errorcluster, "TestCase out"=w427:refnum<class "testcase-CSMBroadcast.lvclass">)  [unwired: 8 in]
    }
  }
  "error out" <- w4
  "TestCase out" <- w2
